vi "WLAN_SuperposedFrameBuild_V3.vi"(4 "Modulation parameter LP":T1, 6 "OFDMON":bool, 7 "Alpha":dbl min=0.0 max=1.0 step=0.05 format="%#_13g", 8 "error in (no error)":errorcluster, 9 "data in 2":i8[](array[numeric]) caption="input bit stream", 10 "Modulation parameter HP":T1, 11 "data in":i8[](array[numeric]) caption="input bit stream") -> (0 "error out":errorcluster, 3 "output array":cdb[](array[numeric]))   [LabVIEW 2022 SP3]
panel:
  out "symbols":cdb[](array[numeric])
  out "x+y":cdb[](array[numeric])
  out "output bit stream 4":i8[](array[numeric])
  out "output bit stream 3":i8[](array[numeric])
  out "subarray 2":i8[](array[numeric])
  out "subarray":i8[](array[numeric])
  out "size(s) 2":i32
  out "size(s) 6":i32
  out "size(s) 5":i32
  out "size(s) 4":i32
  out "size(s) 3":i32
  out "size(s)":i32
  in  "data in 3":i8[](array[numeric]) caption="input bit stream"
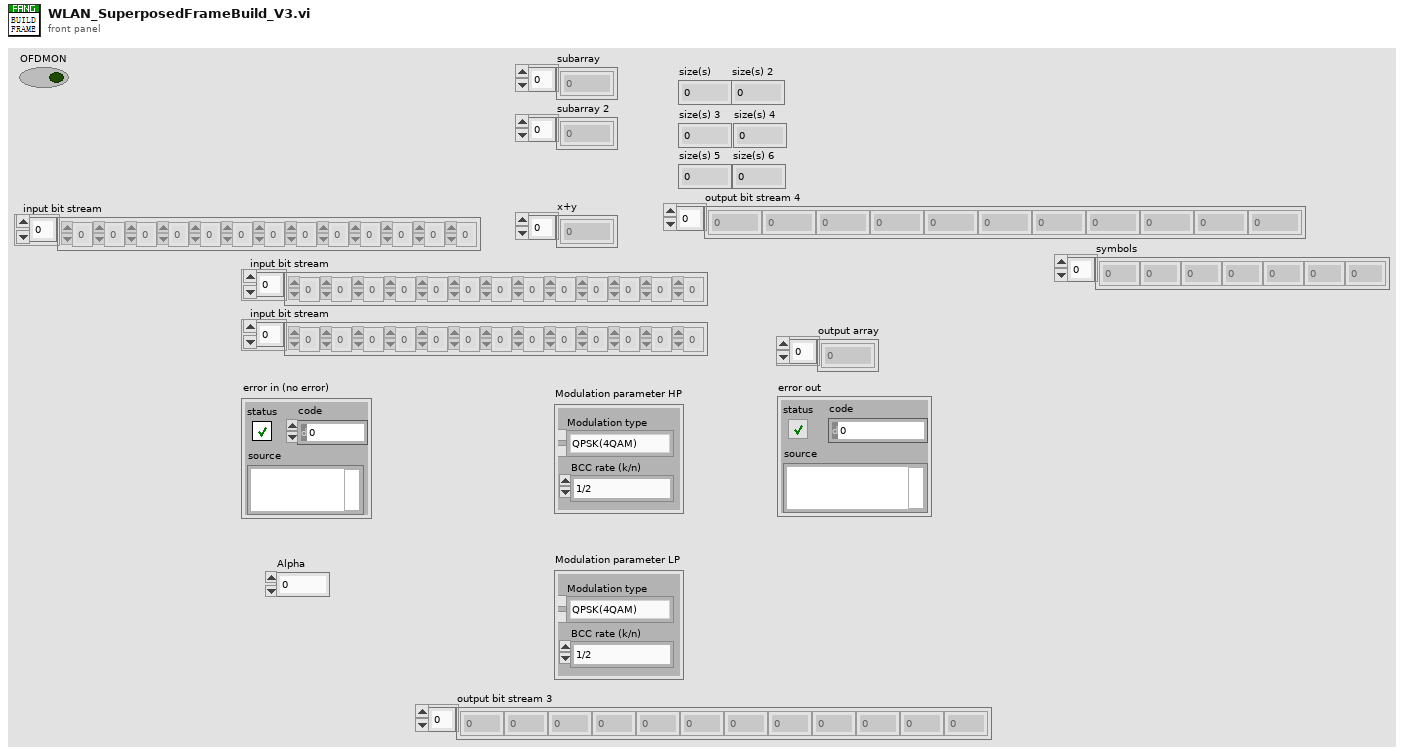
[diagram p1: front panel]
types:
  T1 = cluster{"Modulation type":enum16{"QPSK(4QAM)", "64QAM", "16QAM", "BPSK"}, "BCC rate (k/n)":enum16{"1/2", "2/3", "3/4"}}
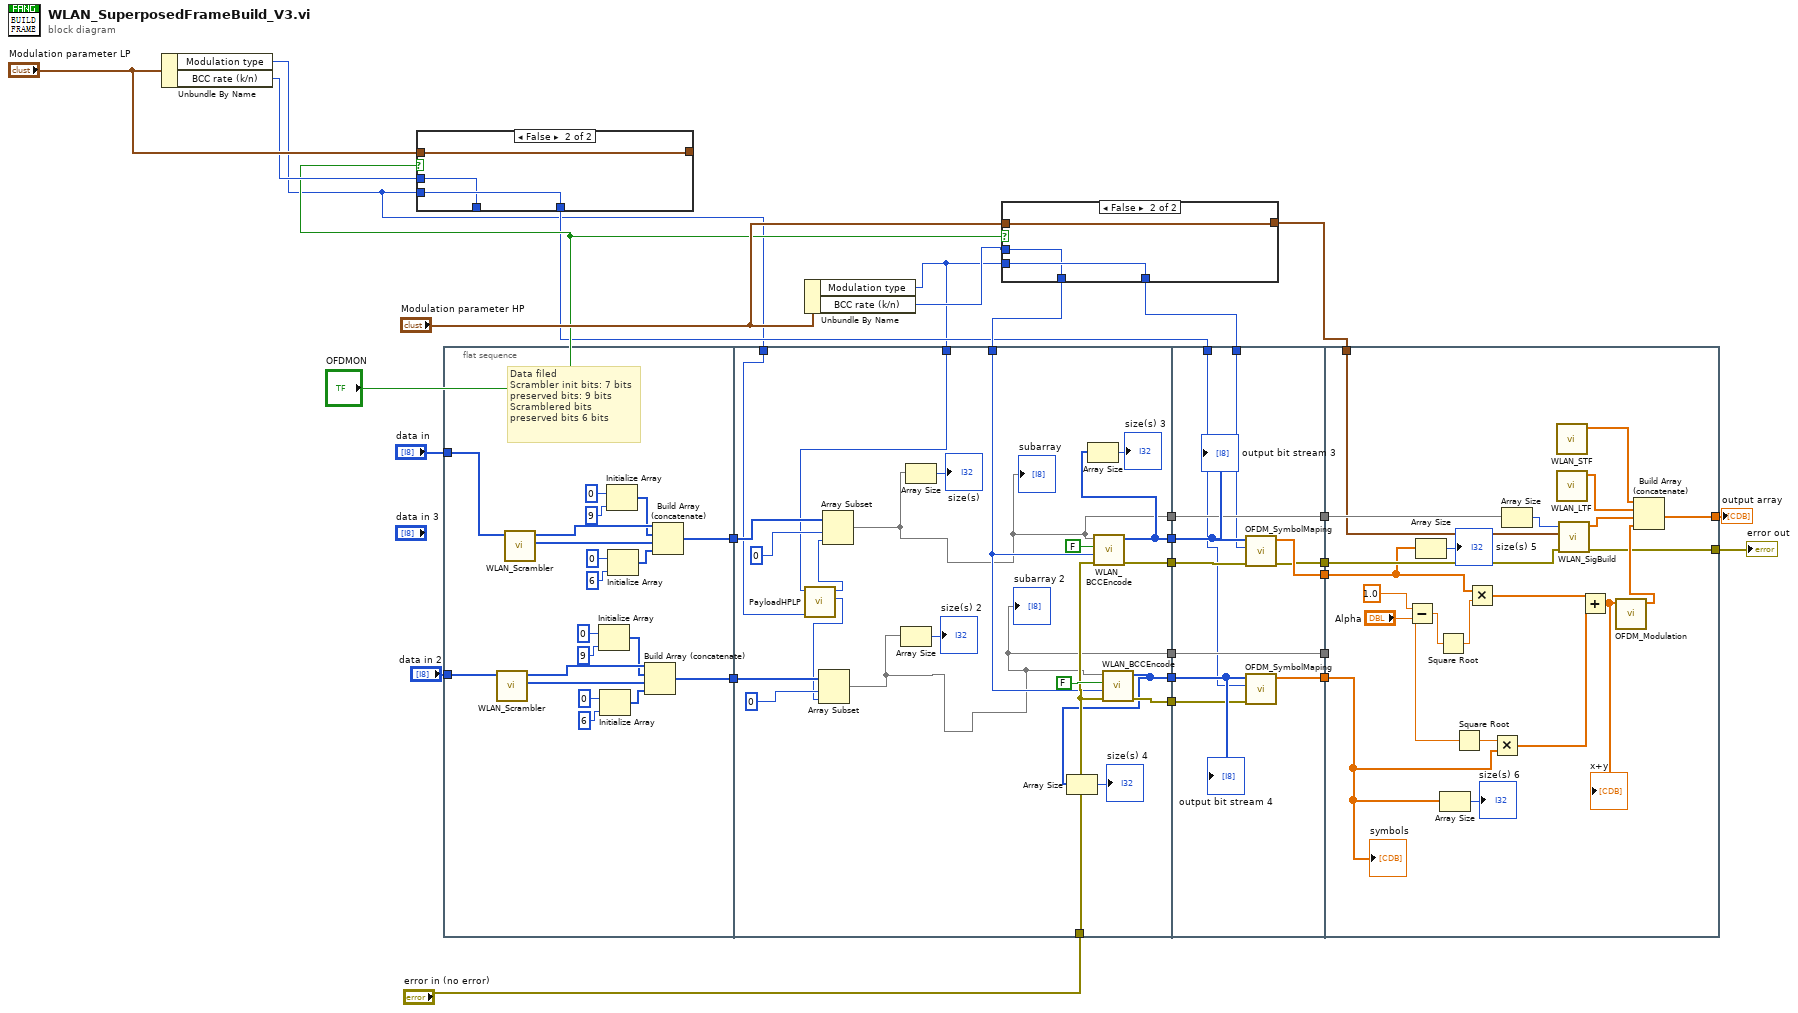
[diagram p0: block diagram]
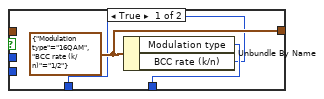
[diagram p2: hidden frame]
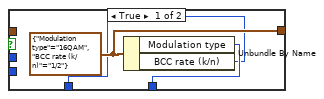
[diagram p3: hidden frame]
diagram:
  n1 = Unbundle By Name("Modulation parameter LP") -> ("Modulation type"=w1:enum16{"QPSK(4QAM)", "64QAM", "16QAM", "BPSK"}, "BCC rate (k/n)"=w5:enum16{"1/2", "2/3", "3/4"})
  n2 = case shown="False" "OFDMON" {
    tunnel: w1 -> [_ w35]
    tunnel: [w32 w35] -> w3
    tunnel: [w31 w34] -> _
    tunnel: "Modulation parameter LP" -> [_ w34]
    tunnel: [w30 w33] -> _
    tunnel: w5 -> [_ w33]
    frame True {
      w31 = T1 {"Modulation type"=enum."16QAM", "BCC rate (k/n)"=enum."1/2"} ("Modulation parameter")
      n3 = Unbundle By Name(w31) -> ("Modulation type"=w32:enum16{"QPSK(4QAM)", "64QAM", "16QAM", "BPSK"}, "BCC rate (k/n)"=w30:enum16{"1/2", "2/3", "3/4"})
    }
    frame False {
    }
  }
  n4 = flat-sequence {
    tunnel: "data in" -> [w47]
    tunnel: [w46] -> w28
    tunnel: "data in 2" -> [w37]
    tunnel: [w36] -> w17
    tunnel: w28 -> [w65]
    tunnel: "error in (no error)" -> [w74]
    tunnel: [w76] -> w26
    tunnel: [w68] -> w25
    tunnel: w8 -> [w73]
    tunnel: [w64] -> w20
    tunnel: w17 -> [w61]
    tunnel: [w60] -> w16
    tunnel: [w67] -> w15
    tunnel: [w72] -> w13
    tunnel: w2 -> [w58]
    tunnel: w1 -> [w57]
    tunnel: w26 -> [w88]
    tunnel: w25 -> [w87]
    tunnel: w11 -> [w79]
    tunnel: [w86] -> w24
    tunnel: [w85] -> w23
    tunnel: w20 -> [w84]
    tunnel: [w84] -> w19
    tunnel: w16 -> [w82]
    tunnel: w15 -> [w83]
    tunnel: [w82] -> w14
    tunnel: w13 -> [w81]
    tunnel: [w80] -> w12
    tunnel: w3 -> [w78]
    tunnel: w10 -> [w108]
    tunnel: w24 -> [w93]
    tunnel: w23 -> [w103]
    tunnel: [w102] -> w22
    tunnel: [w101] -> w21
    tunnel: w19 -> [w110]
    tunnel: w14 -> [_]
    tunnel: w12 -> [w91]
    frame #0 {
      # "Data filed\nScrambler init bits: 7 bits\npreserved bits: 9 bits\nScramblered bits\npreserved bits 6 bits"
      n5 = call "WLAN_Scrambler.vi"("input bit stream"=w37) -> ("scrambled bits"=w41:i8[], "scrambler initial bit"=w45:i8[])  [unwired: 9 in]
      n6 = call "WLAN_Scrambler.vi"("input bit stream"=w47) -> ("scrambled bits"=w51:i8[], "scrambler initial bit"=w55:i8[])  [unwired: 9 in]
      n7 = Initialize Array(i8 0 ("element"), 9 ("dimension size")) -> (w44:i8[])
      n8 = Initialize Array(i8 0 ("element"), 6 ("dimension size")) -> (w38:i8[])
      n9 = Initialize Array(i8 0 ("element"), 9 ("dimension size")) -> (w54:i8[])
      n10 = Initialize Array(i8 0 ("element"), 6 ("dimension size")) -> (w48:i8[])
      n11 = Build Array (concatenate)(w45, w44, w41, w38) -> (w36:i8[])
      n12 = Build Array (concatenate)(w55, w54, w51, w48) -> (w46:i8[])
    }
    frame #1 {
      n13 = call "PayloadHPLP.vi"("Modulation type LP"=w57, "Modulation type HP"=w58) -> ("Payload_LP"=w59:i32, "Payload_HP"=w56:i32)  [unwired: 8 in]
      n14 = Array Subset(array=w61, index=0, length=w59) -> (w60:i8[])
      "subarray 2" <- w60
      n15 = Array Subset(array=w65, index=0, length=w56) -> (w64:i8[])
      "subarray" <- w64
      n16 = Array Size(array=w60) -> (size(s)=→"size(s) 2":i32)
      n17 = Array Size(array=w64) -> (size(s)=→"size(s)":i32)
      n18 = call "WLAN_BCCEncode.vi"("error in (no error)"=w74, "BCC rate (k/n)"=w73, "need add zeros?"=FALSE, "input bit stream"=w64) -> ("error out"=w76:errorcluster, "output bit stream 3"=w68:i8[])  [unwired: 6 in]
      n19 = Array Size(array=w68) -> (size(s)=→"size(s) 3":i32)
      n20 = call "WLAN_BCCEncode.vi"("error in (no error)"=w74, "BCC rate (k/n)"=w73, "need add zeros?"=FALSE, "input bit stream"=w60) -> ("error out"=w72:errorcluster, "output bit stream 3"=w67:i8[])  [unwired: 6 in]
      n21 = Array Size(array=w67) -> (size(s)=→"size(s) 4":i32)
    }
    frame #2 {
      n22 = call "OFDM_SymbolMaping.vi"("error in (no error)"=w88, "Modulation type"=w79, "input bit stream"=w87) -> ("error out"=w85:errorcluster, "symbols"=w86:cdb[])  [unwired: 7 in]
      n23 = call "OFDM_SymbolMaping.vi"("error in (no error)"=w81, "Modulation type"=w78, "input bit stream"=w83) -> ("symbols"=w80:cdb[])  [unwired: 7 in, 1 out]
      "output bit stream 3" <- w87
      "output bit stream 4" <- w83
    }
    frame #3 {
      n24 = Subtract(x=1.0, y="Alpha") -> (x-y=w96:dbl)
      n25 = Array Size(array=w93) -> (size(s)=→"size(s) 5":i32)
      n26 = Square Root(x=w96) -> (sqrt(x)=w98:dbl)
      n27 = Array Size(array=w91) -> (size(s)=→"size(s) 6":i32)
      n28 = Square Root(x="Alpha") -> (sqrt(x)=w99:dbl)
      n29 = Multiply(x=w93, y=w98) -> (x*y=w89:cdb[])
      n30 = Multiply(x=w99, y=w91) -> (x*y=w100:cdb[])
      n31 = Array Size(array=w110) -> (size(s)=w109:i32)
      n32 = call "WLAN_STF.vi"() -> ("STF"=w104:cdb[])  [unwired: 11 in]
      n33 = call "WLAN_LTF.vi"() -> ("LTF"=w105:cdb[])  [unwired: 11 in]
      n34 = call "WLAN_SigBuild.vi"("Data bit length"=w109, "Modulation parameter"=w108, "error in (no error)"=w103) -> ("symbols"=w106:cdb[], "error out"=w102:errorcluster)  [unwired: 6 in]
      n35 = Add(x=w89, y=w100) -> (x+y=w94:cdb[])
      "x+y" <- w94
      n36 = call "OFDM_Modulation.vi"("Input sequence"=w94) -> ("Output sequence"=w107:cdb[])  [unwired: 10 in]
      n37 = Build Array (concatenate)(w104, w105, w106, w107) -> (w101:cdb[])
      "symbols" <- w91
    }
  }
  n38 = Unbundle By Name("Modulation parameter HP") -> ("Modulation type"=w2:enum16{"QPSK(4QAM)", "64QAM", "16QAM", "BPSK"}, "BCC rate (k/n)"=w7:enum16{"1/2", "2/3", "3/4"})
  n39 = case shown="False" "OFDMON" {
    tunnel: w2 -> [_ w116]
    tunnel: [w113 w116] -> w11
    tunnel: [w112 w115] -> w10
    tunnel: "Modulation parameter HP" -> [_ w115]
    tunnel: [w111 w114] -> w8
    tunnel: w7 -> [_ w114]
    frame True {
      w112 = T1 {"Modulation type"=enum."16QAM", "BCC rate (k/n)"=enum."1/2"} ("Modulation parameter")
      n40 = Unbundle By Name(w112) -> ("Modulation type"=w113:enum16{"QPSK(4QAM)", "64QAM", "16QAM", "BPSK"}, "BCC rate (k/n)"=w111:enum16{"1/2", "2/3", "3/4"})
    }
    frame False {
    }
  }
  "output array" <- w21
  "error out" <- w22
